vi "Set Tree Symbols.vi"(8 "error in":errorcluster, 10 "Tag":string, 11 "CtlRef":refnum<vi>) -> (0 "error out":errorcluster)   [LabVIEW 2025, in "Protection and Counter Addon System Explorer.lvlib"]
uses:
  Protection and Counter Addon System Explorer.lvlib
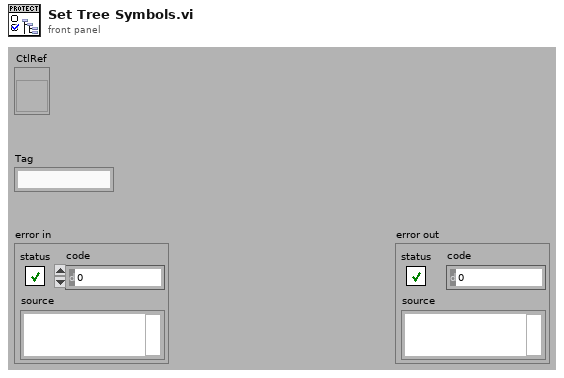
[diagram p1: front panel]
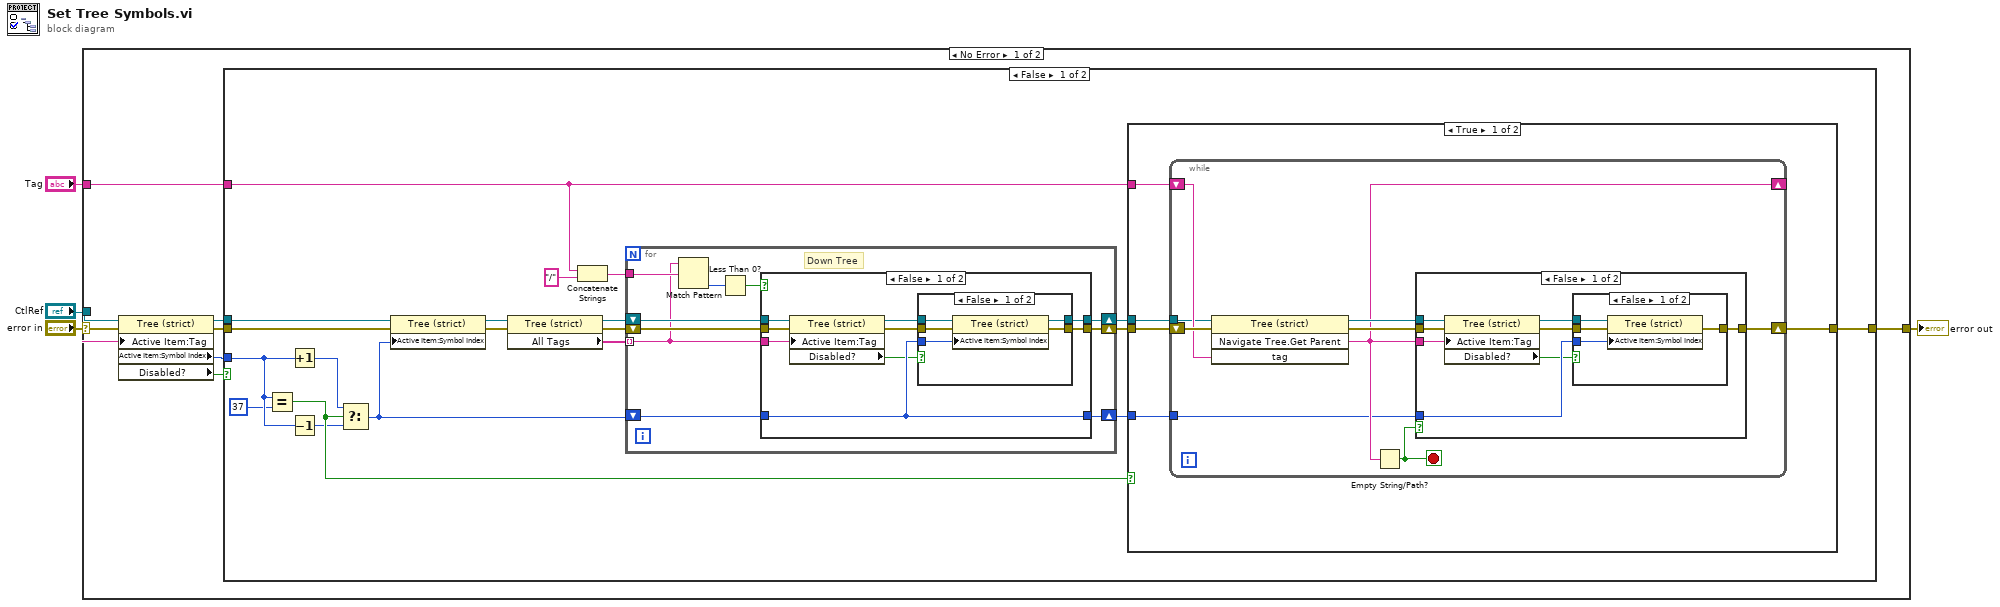
[diagram p0: block diagram]
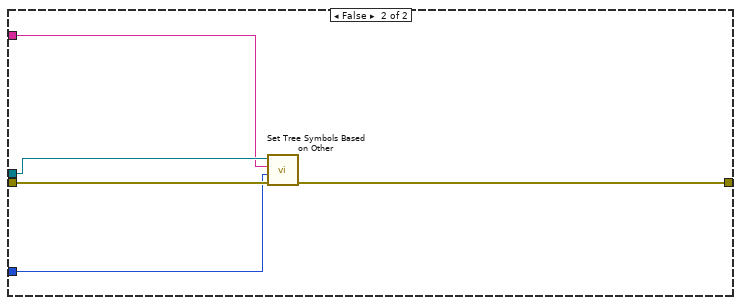
[diagram p4: hidden frame]
diagram:
  n1 = case shown="No Error" "error in" {
    selector: "error in" -> [w6 w96]
    tunnel: [w12 w96] -> w4
    tunnel: "Tag" -> [w11 _]
    tunnel: "CtlRef" -> [w10 _]
    frame No Error {
      n2 = property class="Tree (strict)"(reference=w10, error in=w6, "Active Item:Tag"=w11) -> (reference out=w8:refnum<vi>, error out=w9:errorcluster, "Active Item:Symbol Index"=w7:i32, "Disabled?"=w5:bool)
      n3 = case shown="False" w5 {
        tunnel: [w31 w95] -> w12
        tunnel: w11 -> [w29 _]
        tunnel: w9 -> [w18 w95]
        tunnel: w8 -> [w17 _]
        tunnel: w7 -> [w15 _]
        frame False {
          n4 = Equal?(x=w15, y=37 ("Active Item:Symbol Index")) -> (x = y?=w26:bool)
          n5 = Increment(x=w15) -> (x+1=w14:i32)
          n6 = Decrement(x=w15) -> (x-1=w16:i32)
          n7 = Select(t=w14, s=w26, f=w16) -> (s? t:f=w27:i32)
          n8 = property class="Tree (strict)"(reference=w17, error in=w18, "Active Item:Symbol Index"=w27) -> (reference out=w19:refnum<vi>, error out=w20:errorcluster)
          n9 = property class="Tree (strict)"(reference=w19, error in=w20) -> (reference out=w22:refnum<vi>, error out=w21:errorcluster, "All Tags"=w25:string[])
          n10 = Concatenate Strings(w29, "/" ("string")) -> (w24:string)
          n11 = for {
            tunnel: w24 -> [w75]
            tunnel: w25 -> [w68] mode=indexing
            shift-right: [w71] -> w28
            shift-left: w21 -> [w70]
            shift-right: [w67] -> w30
            shift-left: w22 -> [w69]
            shift-right: [w66] -> w32
            shift-left: w27 -> [w72]
            # "Down Tree"
            n12 = Match Pattern(string=w68, regular expression=w75) -> (offset past match=w74:i32)  [unwired: 1 in, 3 out]
            n13 = Less Than 0?(x=w74) -> (x < 0?=w73:bool)
            n14 = case shown="False" w73 {
              tunnel: w70 -> [w83 w94]
              tunnel: w69 -> [w84 w93]
              tunnel: w68 -> [w82 _]
              tunnel: w72 -> [w77 w92]
              tunnel: [w78 w94] -> w71
              tunnel: [w79 w93] -> w67
              tunnel: [w77 w92] -> w66
              frame False {
                n15 = property class="Tree (strict)"(reference=w84, error in=w83, "Active Item:Tag"=w82) -> (reference out=w80:refnum<vi>, error out=w81:errorcluster, "Disabled?"=w76:bool)
                n16 = case shown="False" w76 {
                  tunnel: w81 -> [w89 w90]
                  tunnel: w80 -> [w88 w91]
                  tunnel: [w87 w91] -> w79
                  tunnel: [w86 w90] -> w78
                  tunnel: w77 -> [w85 _]
                  frame False {
                    n17 = property class="Tree (strict)"(reference=w88, error in=w89, "Active Item:Symbol Index"=w85) -> (reference out=w87:refnum<vi>, error out=w86:errorcluster)
                  }
                  frame True {
                  }
                }
              }
              frame True {
              }
            }
          }
          n18 = case shown="True" w26 {
            tunnel: w28 -> [w37 w64]
            tunnel: w29 -> [w36 w62]
            tunnel: w30 -> [w35 w63]
            tunnel: [w34 w65] -> w31
            tunnel: w32 -> [w33 w61]
            frame True {
              n19 = while {
                tunnel: w35 -> [w44]
                shift-right: [w39] -> w34
                shift-left: w37 -> [w46]
                shift-right: [w41] -> _
                shift-left: w36 -> [w45]
                tunnel: w33 -> [w40]
                stop <- w38 stop-if-true
                n20 = invoke on="Invoke Node" class="Tree (strict)" method="Navigate Tree.Get Parent"(reference=w44, error in=w46, "tag"=w45) -> (reference out=w43:refnum<vi>, error out=w42:errorcluster, "Navigate Tree:Get Parent"=w41:string)  [unwired: 1 in, 1 out]
                n21 = Empty String/Path?(string/path=w41) -> (empty?=w38:bool)
                n22 = case shown="False" w38 {
                  tunnel: w42 -> [w53 w60]
                  tunnel: w43 -> [w54 _]
                  tunnel: w41 -> [w52 _]
                  tunnel: w40 -> [w48 _]
                  tunnel: [w49 w60] -> w39
                  frame False {
                    n23 = property class="Tree (strict)"(reference=w54, error in=w53, "Active Item:Tag"=w52) -> (reference out=w50:refnum<vi>, error out=w51:errorcluster, "Disabled?"=w47:bool)
                    n24 = case shown="False" w47 {
                      tunnel: w51 -> [w58 w59]
                      tunnel: w50 -> [w57 _]
                      tunnel: [w56 w59] -> w49
                      tunnel: w48 -> [w55 _]
                      frame False {
                        n25 = property class="Tree (strict)"(reference=w57, error in=w58, "Active Item:Symbol Index"=w55) -> (error out=w56:errorcluster)  [unwired: 1 out]
                      }
                      frame True {
                      }
                    }
                  }
                  frame True {
                  }
                }
              }
            }
            frame False {
              n26 = call "Set Tree Symbols Based on Other.vi"("error in (no error)"=w64, "Numeric"=w61, "Tag"=w62, "TreeControl in"=w63) -> ("error out"=w65:errorcluster)  [unwired: 7 in]
            }
          }
        }
        frame True {
        }
      }
    }
    frame Error {
    }
  }
  "error out" <- w4
